vi "student_key fob.vi"(11 "wavefor":waveform(cdb)) -> (3 "Button Pressed":i32)   [LabVIEW 2015]
uses:
  <vilib>/measure/mascope.llb/Pulse Measurements 1 chan.vi
  <vilib>/Analysis/2dsp.llb/1D Cross Correlation (DBL).vi
  <vilib>/measure/NI_MAPro.lvlib
  <vilib>/Analysis/NI_AALPro.lvlib
panel:
  out "encoded signal":i16[](graph)
  out "number":u32
  out "message":bool[](array[boolean])
  out "0, 1":i16[](array[numeric])
  out "pulse stream":bool[](array[boolean])
  out "Duration":dbl[](graph)
  out "After ID":dbl[](graph)
  out "Envelope":dbl[](graph)
  out "IQ graph":dbl[](graph)
  out "sample rate":dbl
  in  "Integration Time (samples)":dbl=9.0
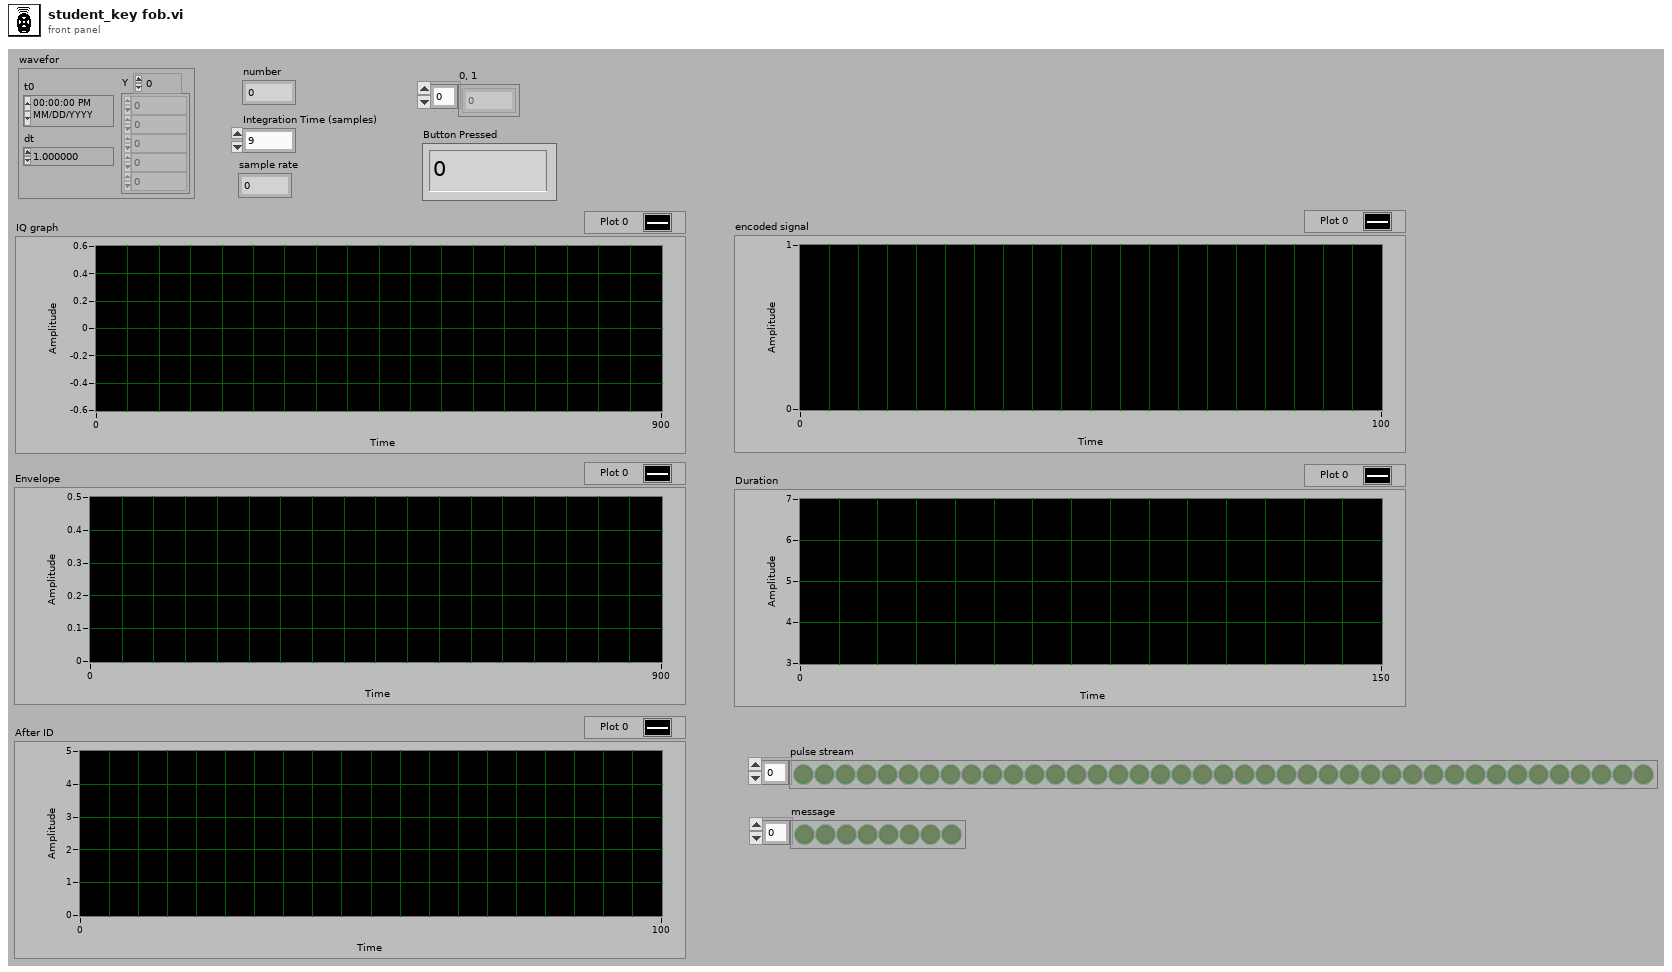
[diagram p1: front panel]
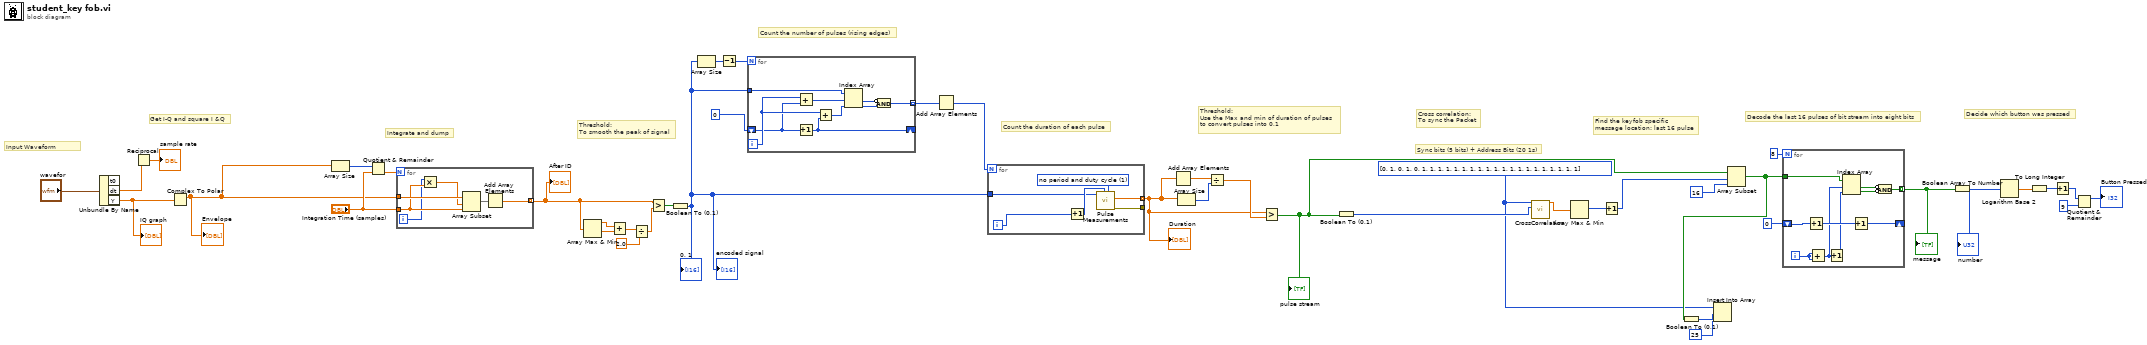
[diagram p0: block diagram]
diagram:
  w1 = i16[] [0, 1, 0, 1, 0, 1, 1, 1, 1, 1, 1, 1, 1, 1, 1, 1, 1, 1, 1, 1, 1, 1, 1, 1, 1] ("0, 1")
  # "Threshold:\nUse the Max and min of duration of pulses \nto convert pulses into 0,1"
  # "Decide which button was pressed"
  # "Decode the last 16 pulses of bit stream into eight bits"
  # "Cross correlation:\nTo sync the Packet"
  # "Count the duration of each pulse"
  # "Threshold:\nTo smooth the peak of signal"
  # "Input Waveform"
  # "Sync bits (5 bits) + Address Bits (20 1s)"
  # "Count the number of pulses (rising edges)"
  # "Find the keyfob specific\nmessage location: last 16 pulse"
  # "Integrate and dump"
  # "Get I-Q and square I &Q"
  n1 = Unbundle By Name("wavefor") -> ("dt"=w37:dbl, "Y"=w35:cdb[])  [unwired: 1 out]
  "IQ graph" <- w35
  n2 = Reciprocal(x=w37) -> (1/x=→"sample rate":dbl)
  n3 = Complex To Polar(r * e^(i*theta)=w35) -> (r=w34:dbl[])  [unwired: 1 out]
  "Envelope" <- w34
  n4 = Array Size(array=w34) -> (size(s)=w44:i32)
  n5 = Quotient & Remainder(x=w44, y="Integration Time (samples)") -> (floor(x/y)=w43:dbl)  [unwired: 1 out]
  n6 = for {
    N: w43 -> [_]
    tunnel: "Integration Time (samples)" -> [w49]
    tunnel: w34 -> [w50]
    tunnel: [w46] -> w27 mode=indexing
    i -> [w45]
    n7 = Multiply(x=w45, y=w49) -> (x*y=w48:dbl)
    n8 = Array Subset(array=w50, index=w48, length=w49) -> (w47:dbl[])
    n9 = Add Array Elements(numeric array=w47) -> (sum=w46:dbl)
  }
  "After ID" <- w27
  n10 = Array Max & Min(array=w27) -> (max value=w33:dbl, min value=w32:dbl)  [unwired: 2 out]
  n11 = Add(x=w33, y=w32) -> (x+y=w31:dbl)
  n12 = Divide(x=w31, y=2.0) -> (x/y=w28:dbl)
  n13 = Greater?(x=w27, y=w28) -> (0:w29:bool[])
  n14 = Boolean To (0,1)(Boolean=w29) -> (0, 1=w5:i16[])
  "0, 1" <- w5
  "encoded signal" <- w5
  n15 = Array Size(array=w5) -> (size(s)=w40:i32)
  n16 = Decrement(x=w40) -> (x-1=w39:i32)
  n17 = for {
    N: w39 -> [_]
    shift-right: [w56] -> _
    shift-left: 0 -> [w57]
    tunnel: [w59] -> w25 mode=indexing
    tunnel: w5 -> [w53]
    i -> [w58]
    n18 = Add(x=w58, y=w57) -> (x+y=w55:i32)
    n19 = Increment(x=w57) -> (x+1=w56:i32)
    n20 = Add(x=w58, y=w56) -> (x+y=w54:i32)
    n21 = Index Array(array=w53, index #1=w55, index #2=w54) -> (element #1=w52:i16, element #2=w51:i16)
    n22 = Compound Arithmetic op=AND(invert w52, w51) -> (w59:i16)
  }
  n23 = Add Array Elements(numeric array=w25) -> (sum=w24:i16)
  n24 = for {
    N: w24 -> [_]
    tunnel: w5 -> [w62]
    tunnel: [w61] -> _
    tunnel: [w60] -> w20 mode=indexing
    i -> [w63]
    w65 = u16 1 items=["all", "no period and duty cycle"] ("export mode")
    n25 = Increment(x=w63) -> (x+1=w64:i32)
    n26 = call-poly <vilib>:"Pulse Measurements.vi"("export mode"=w65, "pulse number (1)"=w64, "signal in"=w62) -> ("error out"=w61:errorcluster, "pulse duration"=w60:dbl)  [unwired: 4 in, 3 out]
  }
  "Duration" <- w20
  n27 = Add Array Elements(numeric array=w20) -> (sum=w23:dbl)
  n28 = Array Size(array=w20) -> (size(s)=w22:i32)
  n29 = Divide(x=w23, y=w22) -> (x/y=w21:dbl)
  n30 = Greater?(x=w20, y=w21) -> (0:w14:bool[])
  "pulse stream" <- w14
  n31 = Boolean To (0,1)(Boolean=w14) -> (0, 1=w19:i16[])
  n32 = call-poly <vilib>:"CrossCorrelation.vi"("Y"=w19, "X"=w1) -> ("Rxy"=w18:dbl[])  [unwired: 8 in, 1 out]
  n33 = Array Max & Min(array=w18) -> (max index (indices)=w16:i32)  [unwired: 3 out]
  n34 = Increment(x=w16) -> (x+1=w15:i32)
  n35 = Array Subset(array=w14, index=w15, length=16) -> (w3:bool[])
  n36 = Boolean To (0,1)(Boolean=w3) -> (0, 1=w4:i16[])
  n37 = Insert Into Array(array=w1, index=25, new element=w4) -> ()  [unwired: 1 out]
  n38 = for {
    N: 8 -> [_]
    shift-right: [w71] -> _
    shift-left: 0 ("x") -> [w75]
    tunnel: [w73] -> w12 mode=indexing
    tunnel: w3 -> [w68]
    i -> [w72]
    n39 = Increment(x=w75) -> (x+1=w74:i32)
    n40 = Add(x=w72, y=w72) -> (x+y=w69:i32)
    n41 = Increment(x=w69) -> (x+1=w70:i32)
    n42 = Index Array(array=w68, index #1=w69, index #2=w70) -> (element #1=w67:bool, element #2=w66:bool)
    n43 = Increment(x=w74) -> (x+1=w71:i32)
    n44 = Compound Arithmetic op=AND(invert w67, invert w66) -> (w73:bool)
  }
  "message" <- w12
  n45 = Boolean Array To Number(Boolean array=w12) -> (number=w10:u32)
  "number" <- w10
  n46 = Logarithm Base 2(1:w10) -> (0:w11:dbl)
  n47 = To Long Integer(number=w11) -> (32bit integer=w9:i32)
  n48 = Increment(x=w9) -> (x+1=w8:i32)
  n49 = Quotient & Remainder(x=w8, y=9) -> (x-y*floor(x/y)=→"Button Pressed":i32)  [unwired: 1 out]
